vi "set first wppos.vi"(8 "error in (no error)":errorcluster, 11 "S4ICS in":refnum<class "S4ICS.lvclass">) -> (0 "error out":errorcluster, 3 "S4ICS out":refnum<class "S4ICS.lvclass">)   [LabVIEW 2018, in "S4ICS.lvclass"]
uses:
  S4ICS.lvclass
  S4ICS.lvclass/S4ICS.ctl
  Mechanism/Mechanism.lvclass
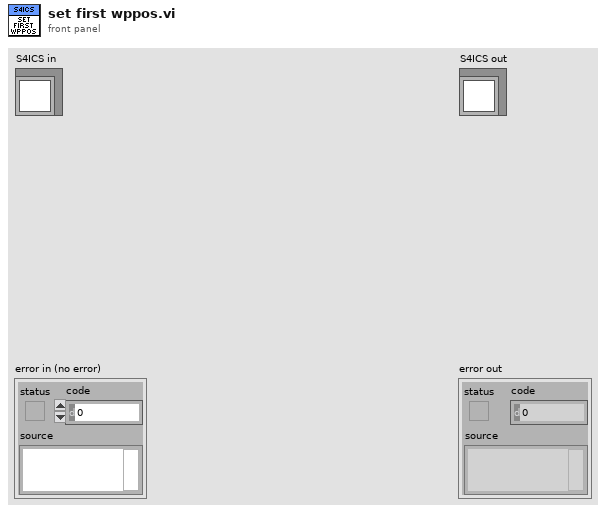
[diagram p1: front panel]
types:
  T1 = cluster{"mode":string, "condition":string, "position":string, "pos_name":string, "pos_id":string}
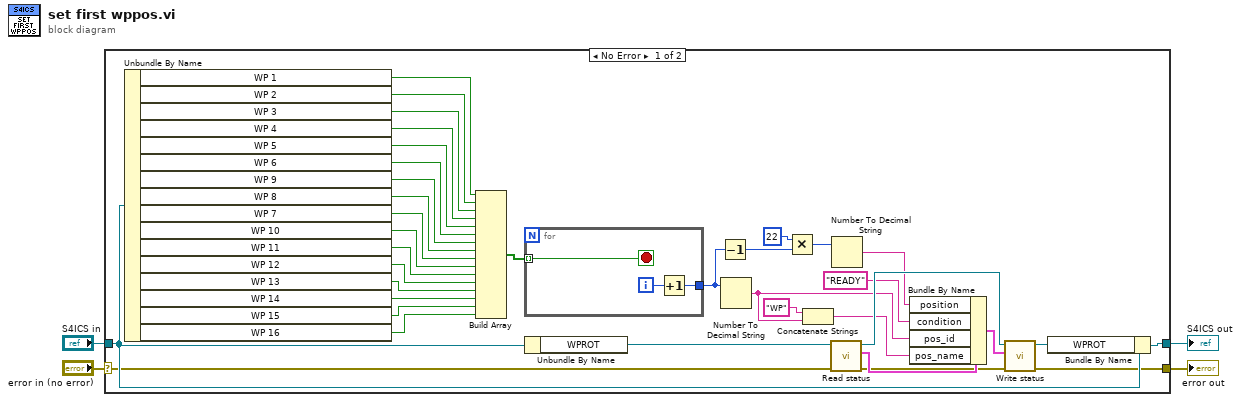
[diagram p0: block diagram]
diagram:
  n1 = case shown="No Error" "error in (no error)" {
    selector: "error in (no error)" -> [w13 w45]
    tunnel: [w11 w45] -> w3
    tunnel: [w24 w44] -> w1
    tunnel: "S4ICS in" -> [w22 w44]
    frame No Error {
      n2 = Unbundle By Name(w22) -> ("WP 1"=w40:bool, "WP 2"=w39:bool, "WP 3"=w38:bool, "WP 4"=w37:bool, "WP 5"=w36:bool, "WP 6"=w35:bool, "WP 9"=w34:bool, "WP 8"=w33:bool, "WP 7"=w32:bool, "WP 10"=w31:bool, "WP 11"=w30:bool, "WP 12"=w29:bool, "WP 13"=w28:bool, "WP 14"=w27:bool, "WP 15"=w26:bool, "WP 16"=w25:bool)
      n3 = Build Array(w40, w39, w38, w37, w36, w35, w34, w33, w32, w31, w30, w29, w28, w27, w26, w25) -> (w23:bool[])
      n4 = for {
        tunnel: w23 -> [w43] mode=indexing
        tunnel: [w41] -> w5
        i -> [w42]
        stop <- w43 stop-if-true
        n5 = Increment(x=w42) -> (x+1=w41:i32)
      }
      n6 = Unbundle By Name(w22) -> ("WPROT"=w20:refnum<class "Mechanism.lvclass">)
      n7 = Decrement(x=w5) -> (x-1=w10:i32)
      n8 = Number To Decimal String(number=w5) -> (decimal integer string=w6:string)  [unwired: 1 in]
      n9 = Multiply(x=22, y=w10) -> (x*y=w8:i32)
      n10 = Concatenate Strings("WP" ("condition"), w6) -> (w14:string)
      n11 = call-dynamic "Read status.vi"("error in (no error)"=w13, "Mechanism in"=w20) -> ("error out"=w12:errorcluster, "status"=w18:T1, "Mechanism out"=w19:refnum<class "Mechanism.lvclass">)  [unwired: 7 in]
      n12 = Number To Decimal String(number=w8) -> (decimal integer string=w7:string)  [unwired: 1 in]
      n13 = Bundle By Name(cluster=w18, "position"=w7, "condition"="READY", "pos_id"=w6, "pos_name"=w14) -> (w17:T1)
      n14 = call-dynamic "Write status.vi"("error in (no error)"=w12, "status"=w17, "Mechanism in"=w19) -> ("error out"=w11:errorcluster, "Mechanism out"=w21:refnum<class "Mechanism.lvclass">)  [unwired: 7 in]
      n15 = Bundle By Name(cluster=w22, "WPROT"=w21) -> (w24:refnum<class "S4ICS.lvclass">)
    }
    frame Error {
    }
  }
  "error out" <- w3
  "S4ICS out" <- w1
